vi "Wave forms.vi"() -> ()   [LabVIEW 2024]
panel:
  in  "Test Names":string[](array[string])
  out "Array":refnum<vi>[](array[refnum])
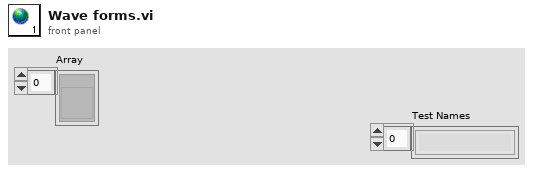
[diagram p1: front panel]
diagram:
